vi "initialize - lan.vi"(8 "error in (no error)":errorcluster, 10 "controller index(0)":u32, 11 "ip":string) -> (0 "error out":errorcluster, 3 "channel handle":u16 format="%x")   [LabVIEW 2024, in "atsj peakcan basic.lvlib"]
doc: "Initializes a PCAN LAN bus (channel) with bitrate adaptation enabled (automatic bitrate selection). This VI supports initialization of both Classical CAN and CAN FD devices.\n\nCopyright (c) 2025 ATSJ (www.atsj.eu)"
uses:
  atsj peakcan basic.lvlib
  bitrate.ctl
  bitrate parameters.ctl
  clock frequency.ctl
  fd bitrate.ctl
  device type.ctl
  get channel handle - by device controller index.vi
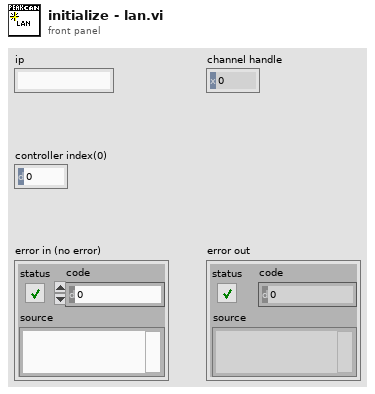
[diagram p1: front panel]
types:
  T1 = typedef "atsj peakcan basic.lvlib/device type.ctl" = enum8{"ISA", "DNG", "PCI", "USB", "PCC", "LAN"}
  T2 = typedef "atsj peakcan basic.lvlib/bitrate.ctl" = enum16{"RATE_1Mbps", "RATE_800kbps", "RATE_500kbps", "RATE_250kbps", "RATE_125kbps", "RATE_100kbps", "RATE_95kbps", "RATE_83kbps", "RATE_50kbps", "RATE_47kbps", "RATE_33kbps", "RATE_20kbps", "RATE_10kbps", "RATE_5kbps"}
  T3 = typedef "atsj peakcan basic.lvlib/fd bitrate.ctl" = cluster{"clock frequency":T4, "nominal bitrate":T5, "data bitrate":T5}
  T4 = typedef "atsj peakcan basic.lvlib/clock frequency.ctl" = enum16{"CLOCK_80MHz", "CLOCK_60MHz", "CLOCK_40MHz", "CLOCK_30MHz", "CLOCK_24MHz", "CLOCK_20MHz"}
  T5 = typedef "atsj peakcan basic.lvlib/bitrate parameters.ctl" = cluster{"bitrate prescaler":u16, "time segment 1":u16, "time segment 2":u16, "sync jump width":u16}
  T6 = typedef "atsj peakcan basic.lvlib/features.ctl" = cluster{"fd capable":bool, "delay capable":bool, "io capable":bool}
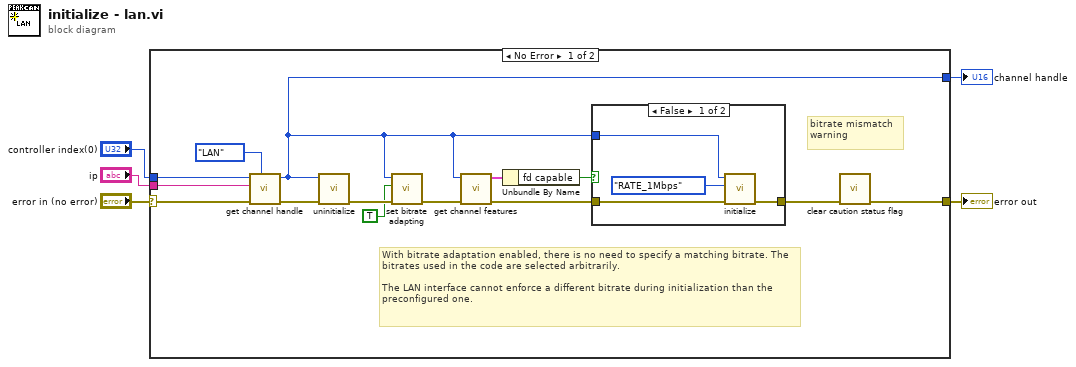
[diagram p0: block diagram]
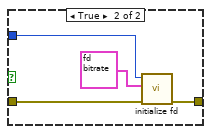
[diagram p2: hidden frame]
diagram:
  n1 = case shown="No Error" "error in (no error)" {
    selector: "error in (no error)" -> [w8 w28]
    tunnel: "ip" -> [w10 _]
    tunnel: "controller index(0)" -> [w9 _]
    tunnel: [w7 w28] -> w2
    tunnel: [w6 _] -> w1
    frame No Error {
      # "bitrate mismatch warning"
      # "With bitrate adaptation enabled, there is no need to specify a matching bitrate. The bitrates used in the code are selected arbitrarily.\n\nThe LAN interface cannot enforce a different bitrate during initialization than the preconfigured one."
      n2 = call-poly "get channel handle.vi"("device type"=device_type."LAN", "error in (no error)"=w8, "ip (\"\")"=w10, "controller index(0)"=w9) -> ("error out"=w12:errorcluster, "channel handle"=w6:u16)  [unwired: 6 in]
      n3 = call "uninitialize.vi"("error in (no error)"=w12, "channel handle (0:all)"=w6) -> ("error out"=w19:errorcluster)  [unwired: 9 in]
      n4 = call "set bitrate adapting.vi"("error in (no error)"=w19, "enable (F)"=TRUE, "channel handle"=w6) -> ("error out"=w15:errorcluster)  [unwired: 8 in]
      n5 = call "get channel features.vi"("error in (no error)"=w15, "channel handle"=w6) -> ("error out"=w17:errorcluster, "features"=w18:T6)  [unwired: 8 in]
      n6 = Unbundle By Name(w18) -> ("fd capable"=w16:bool)
      n7 = case shown="False" w16 {
        tunnel: w17 -> [w23 w27]
        tunnel: w6 -> [w22 w26]
        tunnel: [w21 w25] -> w13
        frame False {
          n8 = call "initialize.vi"("error in (no error)"=w23, "bitrate"=bitrate."RATE_1Mbps", "channel handle"=w22) -> ("error out"=w21:errorcluster)  [unwired: 8 in]
        }
        frame True {
          n9 = call "initialize fd.vi"("error in (no error)"=w27, "bitrate"=T3 {"clock frequency"=enum."CLOCK_80MHz", "nominal bitrate"={"bitrate prescaler"=2, "time segment 1"=63, "time segment 2"=16, "sync jump width"=16}, "data bitrate"={"bitrate prescaler"=2, "time segment 1"=15, "time segment 2"=4, "sync jump width"=4}}, "channel handle"=w26) -> ("error out"=w25:errorcluster)  [unwired: 8 in]
        }
      }
      n10 = call "clear caution status flag.vi"("error in (no error)"=w13) -> ("error out"=w7:errorcluster)  [unwired: 9 in, 1 out]
    }
    frame Error {
    }
  }
  "error out" <- w2
  "channel handle" <- w1
